vi "Async Actor.vi"(10 "Unified Actor":refnum<class "Actor.lvclass">) -> (0 "Error out":errorcluster, 2 "Child Attributes":refnum<class "Attributes.lvclass">)   [LabVIEW 2020, in "jettl.lvlib"]
uses:
  jettl.lvlib
  Actor/Actor.lvclass
  Attributes/Attributes.lvclass
  Async Elements.ctl
  Base Async Elements/Base Async Elements/Base Async Elements.lvclass/Base Async Elements.ctl
  Base Async Elements/Base Async Elements/Base Async Elements.lvclass
  C:/git/jettl/src/jettl/jettl/Async Elements/Async Elements.lvclass
  Actor.vi
  Async Elements/Async Elements.lvclass
  Base Async Elements/Base Async Elements.lvlib
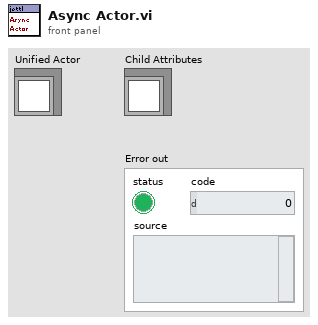
[diagram p1: front panel]
types:
  T1 = typedef "jettl.lvlib/Async Elements.ctl" = cluster{"Attributes":refnum<class "Attributes.lvclass">, "Error":errorcluster}
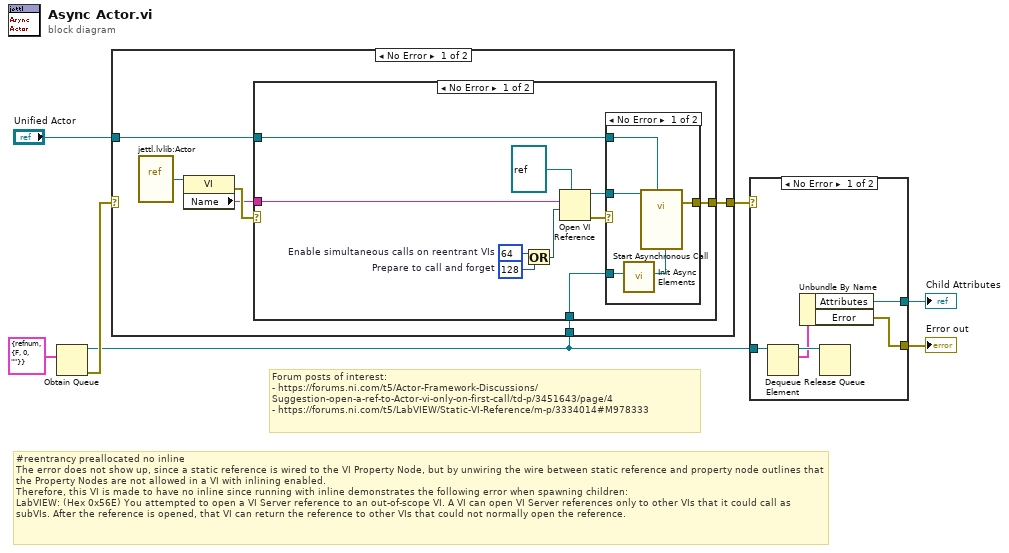
[diagram p0: block diagram]
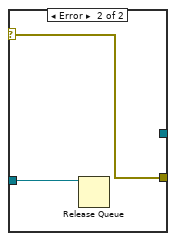
[diagram p5: hidden frame]
diagram:
  # "#reentrancy preallocated no inline\nThe error does not show up, since a static reference is wired to the VI Property Node, but by unwiring the wire between static reference and property node outlines that the Property Nodes are not allowed in a VI with inlining enabled.\nTherefore, this VI is made to have no inline since running with inline demonstrates the following error when spawning children:\nLabVIEW: (Hex 0x56E) You attempted to open a VI Server reference to an out-of-scope VI. A VI can open VI Server references only to other VIs that it could call as subVIs. After the reference is opened, that VI can return the reference to other VIs that could not normally open the reference."
  # "Forum posts of interest:\n- https://forums.ni.com/t5/Actor-Framework-Discussions/Suggestion-open-a-ref-to-Actor-vi-only-on-first-call/td-p/3451643/page/4\n- https://forums.ni.com/t5/LabVIEW/Static-VI-Reference/m-p/3334014#M978333"
  n1 = Obtain Queue(element data type=T1 {"Attributes"=refnum, "Error"={"status"=FALSE, "code"=0, "source"=""}} ("Async Elements")) -> (queue out=w1:refnum<queue>, error out=w3:errorcluster)  [unwired: 4 in, 1 out]
  n2 = case shown="No Error" w3 {
    selector: w3 -> [_ w31]
    tunnel: [w11 w31] -> w7
    tunnel: "Unified Actor" -> [w13 _]
    tunnel: w1 -> [w12 _]
    frame No Error {
      n3 = vi-ref "jettl.lvlib:Actor.vi"() -> (w10:refnum<vi>)
      n4 = property class="VI"(reference=w10) -> (error out=w9:errorcluster, "Name"=w8:string)  [unwired: 1 in, 1 out]
      n5 = case shown="No Error" w9 {
        selector: w9 -> [_ w30]
        tunnel: w13 -> [w23 _]
        tunnel: w12 -> [w22 _]
        tunnel: [w15 w30] -> w11
        tunnel: w8 -> [w14 _]
        frame No Error {
          w18 = 64  # Enable simultaneous calls on reentrant VIs
          w20 = 128  # Prepare to call and forget
          n6 = Or(x=w18, y=w20) -> (x .or. y?=w19:i32)
          n7 = Open VI Reference(type specifier VI Refnum (for type only)=refnum<vi> refnum, vi path=w14, options=w19) -> (vi reference=w17:refnum<vi>, error out=w16:errorcluster)  [unwired: 3 in]
          n8 = case shown="No Error" w16 {
            selector: w16 -> [_ w29]
            tunnel: w23 -> [w28 _]
            tunnel: w22 -> [w27 _]
            tunnel: w17 -> [w25 _]
            tunnel: [w24 w29] -> w15
            frame No Error {
              n9 = call "Init Async Elements.vi"("Async Elements"=w27) -> ("Async Elements"=w26:refnum<class "Async Elements.lvclass">)  [unwired: 10 in]
              n10 = call-by-ref "Start Asynchronous Call"(reference=w25, "Async Elements"=w26, "Actor in"=w28) -> (error out=w24:errorcluster)  [unwired: 9 in, 3 out]
            }
            frame Error {
            }
          }
        }
        frame Error {
        }
      }
    }
    frame Error {
    }
  }
  n11 = case shown="No Error" w7 {
    selector: w7 -> [_ w37]
    tunnel: w1 -> [w36 w38]
    tunnel: [w33 w37] -> w5
    tunnel: [w34 _] -> w4
    frame No Error {
      n12 = Dequeue Element(queue=w36) -> (queue out=w35:refnum<queue>, element=w32:T1)  [unwired: 2 in, 2 out]
      n13 = Unbundle By Name(w32) -> ("Attributes"=w34:refnum<class "Attributes.lvclass">, "Error"=w33:errorcluster)
      n14 = Release Queue(queue=w35) -> ()  [unwired: 2 in, 3 out]
    }
    frame Error {
      n15 = Release Queue(queue=w38) -> ()  [unwired: 2 in, 3 out]
    }
  }
  "Error out" <- w5
  "Child Attributes" <- w4
